vi "Demo Main.vi"   [LabVIEW 2020, in "VolatusDemo.lvlib"]
uses:
  VolatusDemo.lvlib
  DemoApp/DemoApp.lvclass
  C:/dev/lv20CE/relink/lv-volatus/Volatus/App/App.lvclass
  Volatus/Volatus.lvlib
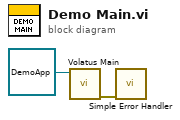
[diagram p0: block diagram]
diagram:
  n1 = call "Volatus Main.vi"("App in"=refnum<class "DemoApp.lvclass"> refnum ("VolatusDemo.lvlib:DemoApp.lvclass")) -> ("error out"=w1:errorcluster)  [unwired: 9 in, 1 out]
  n2 = call <vilib>:"Simple Error Handler.vi"("error in (no error)"=w1) -> ()  [unwired: 4 in, 5 out]
